vi "PicoScope6000aAdvancedTriggerPWQ.vi"(0 "handle in":i16=16384, 1 "Pulse Width Qualifier Settings":T3 {"Pulse Width Type" items=["None", "Less Than", "Greater Than", "In Range", "Out of Range"]}, 2 "Pulse Width Qualifier Trigger Properties":T1={"Channel A Trigger Properties"={"Threshold Mode"=0, "Available"=TRUE, "Direction"=2}, "Channel B Trigger Properties"={"Threshold Mode"=0, "Available"=FALSE, "Direction"=2}, "Channel C Trigger Properties"={"Threshold Mode"=0, "Available"=FALSE, "Direction"=2}, "Channel D Trigger Properties"={"Threshold Mode"=0, "Available"=FALSE, "Direction"=2}, "Channel E Trigger Properties"={"Threshold Mode"=0, "Available"=FALSE, "Direction"=2}, "Channel F Trigger Properties"={"Threshold Mode"=0, "Available"=FALSE, "Direction"=2}, "Channel G Trigger Properties"={"Threshold Mode"=0, "Available"=FALSE, "Direction"=2}, "Channel H Trigger Properties"={"Threshold Mode"=0, "Available"=FALSE, "Direction"=2}, "Port 0 Trigger Properties"={"Threshold Mode"=0, "Available"=FALSE, "Direction"=2}, "Port 1 Trigger Properties"={"Threshold Mode"=0, "Available"=FALSE, "Direction"=2}} {"Port 1 Trigger Properties"."Direction" items=["Rising"=2, "Falling"=3, "Rising Lower"=7, "Above"=0, "Below"=1, "Rising or Falling"=4, "Falling Lower"=8, "Below Lower"=6, "Above Lower"=5]; "Port 1 Trigger Properties"."Threshold Mode" items=["Level", "Window"]; "Port 0 Trigger Properties"."Direction" items=["Rising"=2, "Falling"=3, "Rising Lower"=7, "Above"=0, "Below"=1, "Rising or Falling"=4, "Falling Lower"=8, "Below Lower"=6, "Above Lower"=5]; "Port 0 Trigger Properties"."Threshold Mode" items=["Level", "Window"]; "Channel H Trigger Properties"."Direction" items=["Rising"=2, "Falling"=3, "Rising Lower"=7, "Above"=0, "Below"=1, "Rising or Falling"=4, "Falling Lower"=8, "Below Lower"=6, "Above Lower"=5]; "Channel H Trigger Properties"."Threshold Mode" items=["Level", "Window"]; "Channel G Trigger Properties"."Direction" items=["Rising"=2, "Falling"=3, "Rising Lower"=7, "Above"=0, "Below"=1, "Rising or Falling"=4, "Falling Lower"=8, "Below Lower"=6, "Above Lower"=5]; "Channel G Trigger Properties"."Threshold Mode" items=["Level", "Window"]; "Channel F Trigger Properties"."Direction" items=["Rising"=2, "Falling"=3, "Rising Lower"=7, "Above"=0, "Below"=1, "Rising or Falling"=4, "Falling Lower"=8, "Below Lower"=6, "Above Lower"=5]; "Channel F Trigger Properties"."Threshold Mode" items=["Level", "Window"]; "Channel E Trigger Properties"."Direction" items=["Rising"=2, "Falling"=3, "Rising Lower"=7, "Above"=0, "Below"=1, "Rising or Falling"=4, "Falling Lower"=8, "Below Lower"=6, "Above Lower"=5]; "Channel E Trigger Properties"."Threshold Mode" items=["Level", "Window"]; "Channel D Trigger Properties"."Direction" items=["Rising"=2, "Falling"=3, "Rising Lower"=7, "Above"=0, "Below"=1, "Rising or Falling"=4, "Falling Lower"=8, "Below Lower"=6, "Above Lower"=5]; "Channel D Trigger Properties"."Threshold Mode" items=["Level", "Window"]; "Channel C Trigger Properties"."Direction" items=["Rising"=2, "Falling"=3, "Rising Lower"=7, "Above"=0, "Below"=1, "Rising or Falling"=4, "Falling Lower"=8, "Below Lower"=6, "Above Lower"=5]; "Channel C Trigger Properties"."Threshold Mode" items=["Level", "Window"]; "Channel B Trigger Properties"."Direction" items=["Rising"=2, "Falling"=3, "Rising Lower"=7, "Above"=0, "Below"=1, "Rising or Falling"=4, "Falling Lower"=8, "Below Lower"=6, "Above Lower"=5]; "Channel B Trigger Properties"."Threshold Mode" items=["Level", "Window"]; "Channel A Trigger Properties"."Direction" items=["Rising"=2, "Falling"=3, "Rising Lower"=7, "Above"=0, "Below"=1, "Rising or Falling"=4, "Falling Lower"=8, "Below Lower"=6, "Above Lower"=5]; "Channel A Trigger Properties"."Threshold Mode" items=["Level", "Window"]}, 11 "error in":errorcluster, 13 "Pulse Width Qualifier Conditions":T2 {"Port 1" items=["Don't Care", "True", "False"]; "Channel H" items=["Don't Care", "True", "False"]; "Channel G" items=["Don't Care", "True", "False"]; "Channel F" items=["Don't Care", "True", "False"]; "Channel E" items=["Don't Care", "True", "False"]; "Aux" items=["Don't Care", "True", "False"]; "Port 0" items=["Don't Care", "True", "False"]; "Channel D" items=["Don't Care", "True", "False"]; "Channel C" items=["Don't Care", "True", "False"]; "Channel B" items=["Don't Care", "True", "False"]; "Channel A" items=["Don't Care", "True", "False"]; "Condition Logic" items=["AND", "OR", "XOR"]}) -> (4 "handle out":i16=16384, 15 "error out":errorcluster)   [LabVIEW 2010]
doc: "This sub VI is an interface for the advanced trigger features of the oscilloscope to support Pulse width qualifier (PWQ)."
uses:
  ps6000a.dll
panel:
  in  "PWQ Info Action XOR":bool=TRUE
  in  "PWQ Info Action OR":bool=TRUE
  # "For Condition Logic Suggested settings;\nFor AND, XOR logic-(parallel triggers)\nUse level-type triggers (Level or Inside/outside Window Triggers)\n\nFor OR logic- (single channel)\nUse edge types (e.g. rising, falling, entering window)"
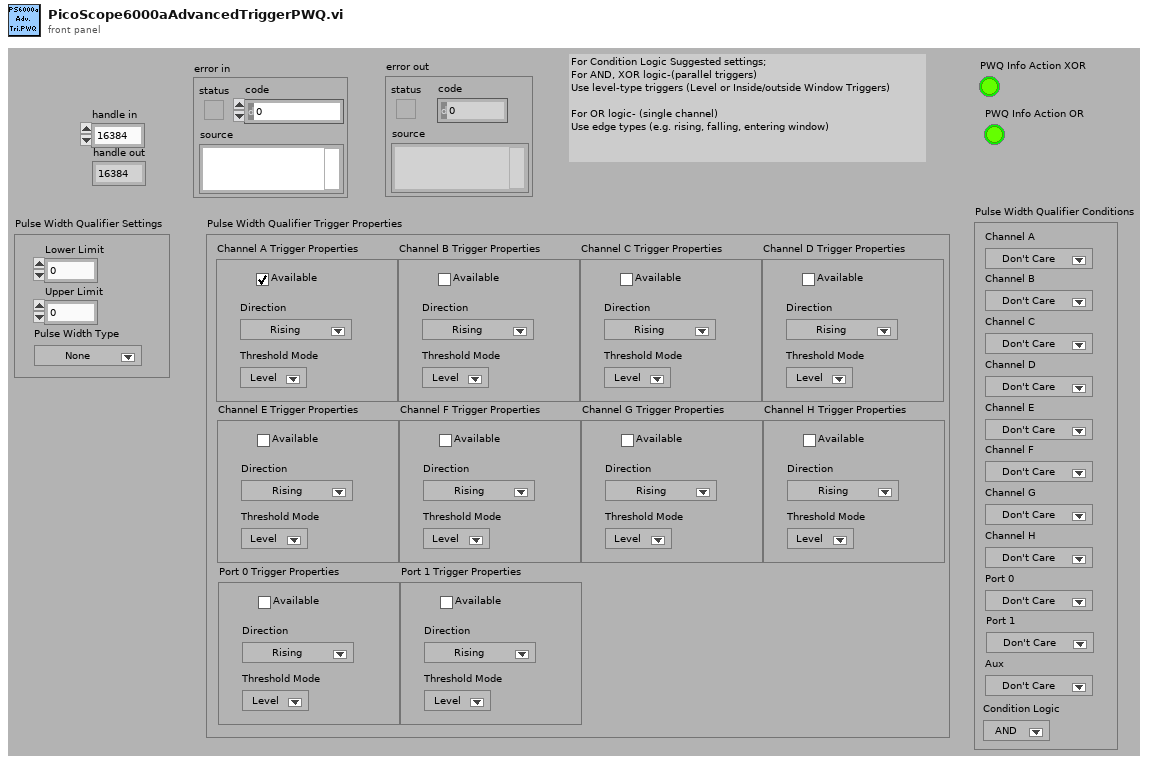
[diagram p1: front panel]
types:
  T1 = cluster{"Channel A Trigger Properties":cluster{"Threshold Mode":i32, "Available":bool, "Direction":u32}, "Channel B Trigger Properties":cluster{"Threshold Mode":i32, "Available":bool, "Direction":u32}, "Channel C Trigger Properties":cluster{"Threshold Mode":i32, "Available":bool, "Direction":u32}, "Channel D Trigger Properties":cluster{"Threshold Mode":i32, "Available":bool, "Direction":u32}, "Channel E Trigger Properties":cluster{"Threshold Mode":i32, "Available":bool, "Direction":u32}, "Channel F Trigger Properties":cluster{"Threshold Mode":i32, "Available":bool, "Direction":u32}, "Channel G Trigger Properties":cluster{"Threshold Mode":i32, "Available":bool, "Direction":u32}, "Channel H Trigger Properties":cluster{"Threshold Mode":i32, "Available":bool, "Direction":u32}, "Port 0 Trigger Properties":cluster{"Threshold Mode":i32, "Available":bool, "Direction":u32}, "Port 1 Trigger Properties":cluster{"Threshold Mode":i32, "Available":bool, "Direction":u32}}
  T2 = cluster{"Channel A":u16, "Channel B":u16, "Channel C":u16, "Channel D":u16, "Channel E":u16, "Channel F":u16, "Channel G":u16, "Channel H":u16, "Port 0":u16, "Port 1":u16, "Aux":u16, "Condition Logic":u16}
  T3 = cluster{"Lower Limit":u32, "Upper Limit":u32, "Pulse Width Type":u32}
  T4 = cluster{"status":bool, "code":u32, "source":string}
  T5 = cluster{"Threshold Mode":i32, "Available":bool, "Direction":u32}[]
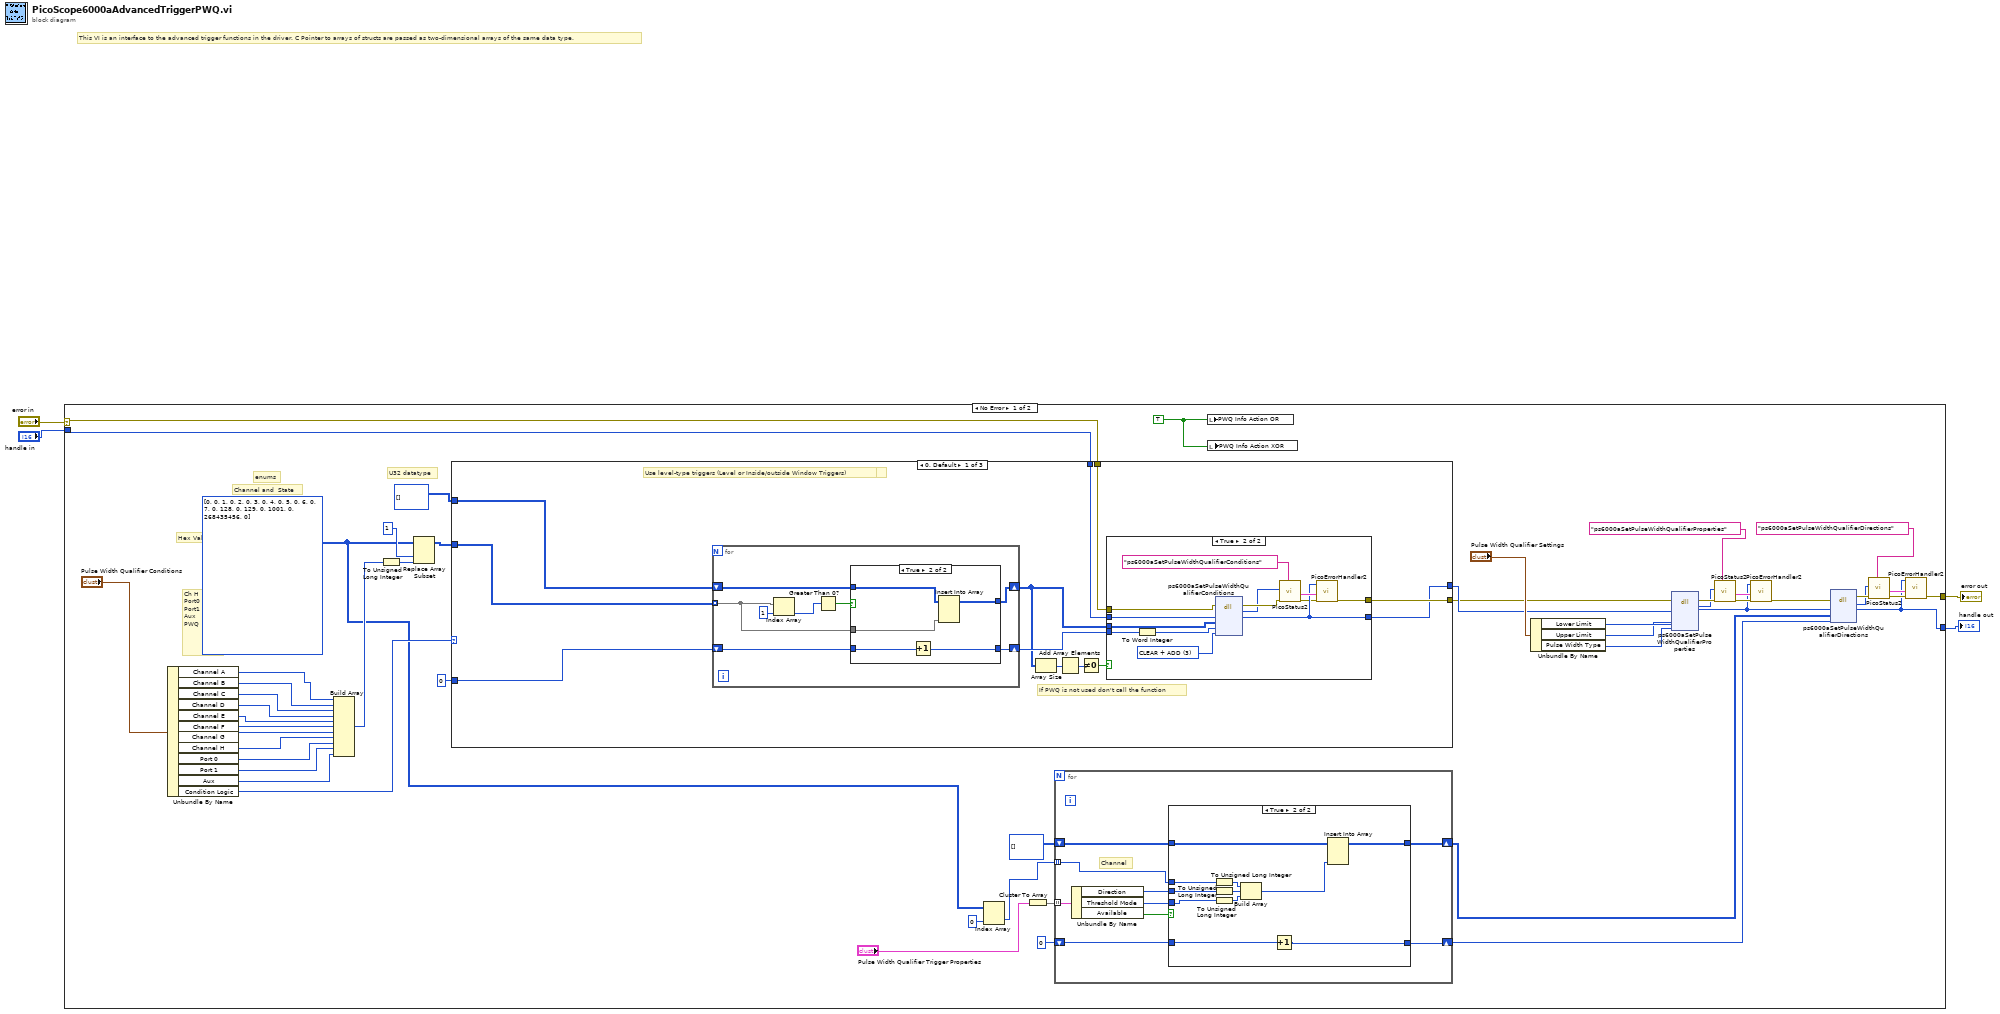
[diagram p0: block diagram]
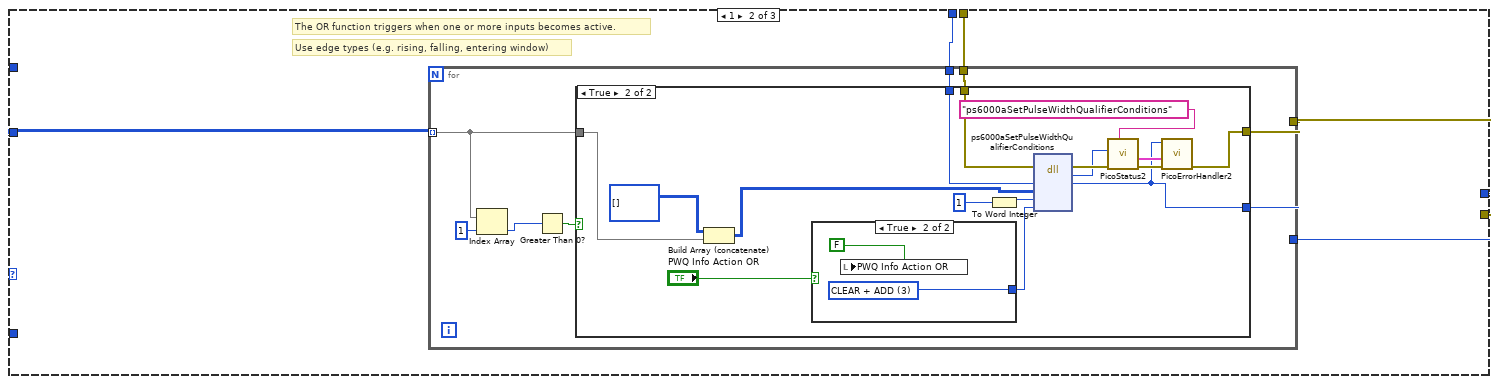
[diagram p5: hidden frame]
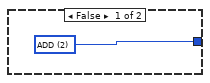
[diagram p7: hidden frame]
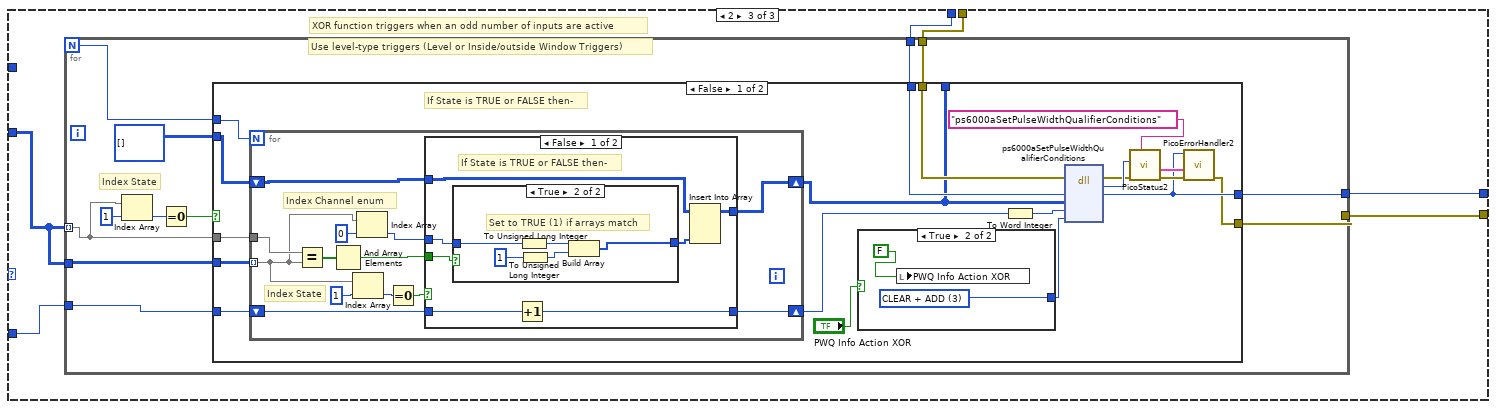
[diagram p8: hidden frame]
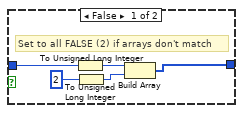
[diagram p9: hidden frame]
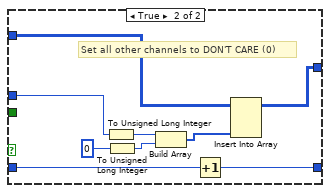
[diagram p10: hidden frame]
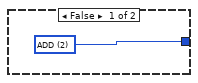
[diagram p11: hidden frame]
diagram:
  # "This VI is an interface to the advanced trigger functions in the driver. C Pointer to arrays of structs are passed as two-dimensional arrays of the same data type."
  n1 = case shown="No Error" "error in" {
    selector: "error in" -> [w20 w236]
    tunnel: "handle in" -> [w19 w237]
    tunnel: [w5 w237] -> w2
    tunnel: [w9 w236] -> w1
    frame No Error {
      w33 = TRUE ("PWQ Info Action XOR")
      w21 = u32[][] [[0, 0], [1, 0], [2, 0], [3, 0], [4, 0], [5, 0], [6, 0], [7, 0], [128, 0], [129, 0], [1001, 0], [268435456, 0]]
      # "U32 datatype"
      # "enums"
      # "Ch H\nPort0\nPort1\nAux\nPWQ"
      # "Channel and  State"
      # "Hex Values"
      n2 = Unbundle By Name("Pulse Width Qualifier Conditions") -> ("Channel A"=w43:u16, "Channel B"=w42:u16, "Channel C"=w41:u16, "Channel D"=w40:u16, "Channel E"=w39:u16, "Channel F"=w38:u16, "Channel G"=w37:u16, "Channel H"=w36:u16, "Port 0"=w35:u16, "Port 1"=w34:u16, "Aux"=w22:u16, "Condition Logic"=w23:u16)
      n3 = Build Array(w43, w42, w41, w40, w39, w38, w37, w36, w35, w34, w22) -> (w54:u16[])
      n4 = To Unsigned Long Integer(number=w54) -> (unsigned 32bit integer=w46:u32[])
      n5 = Replace Array Subset(array=w21, new element=w46, index (col)=1 ("disabled index (col)")) -> (w45:u32[][])  [unwired: 1 in]
      n6 = case shown="0, Default" w23 {
        tunnel: u32[][] [] -> [w89 _ _]
        tunnel: i16 0 -> [w88 _ w154]
        tunnel: w20 -> [w85 w124 w159]
        tunnel: w19 -> [w84 w123 w158]
        tunnel: [w83 w122 w157] -> w47
        tunnel: [w82 w121 w156] -> w48
        tunnel: w45 -> [w86 w120 w155]
        frame 0, Default {
          # "If PWQ is not used don't call the function"
          # "AND function requires both inputs to be active before it will trigger."
          # "Use level-type triggers (Level or Inside/outside Window Triggers)"
          n7 = for {
            shift-right: [w111] -> w87
            shift-left: w88 -> [w110]
            shift-right: [w109] -> w81
            shift-left: w89 -> [w112]
            tunnel: w86 -> [w107] mode=indexing
            n8 = Index Array(array=w107, index=1) -> (element=w106:u32)
            n9 = Greater Than 0?(x=w106) -> (x > 0?=w108:bool)
            n10 = case shown="True" w108 {
              tunnel: w112 -> [w114 w119]
              tunnel: [w114 w118] -> w109
              tunnel: [w113 w117] -> w111
              tunnel: w110 -> [w113 w116]
              tunnel: w107 -> [_ w115]
              frame False {
              }
              frame True {
                n11 = Increment(x=w116) -> (x+1=w117:i16)
                n12 = Insert Into Array(array=w119, new element=w115) -> (w118:u32[][])  [unwired: 2 in]
              }
            }
          }
          n13 = Array Size(array=w81) -> (size(s)=w79:i32[])
          n14 = Add Array Elements(numeric array=w79) -> (sum=w80:i32)
          n15 = Not Equal To 0?(x=w80) -> (x != 0?=w78:bool)
          n16 = case shown="True" w78 {
            tunnel: w87 -> [_ w104]
            tunnel: w85 -> [w91 w103]
            tunnel: w84 -> [w90 w102]
            tunnel: w81 -> [_ w99]
            tunnel: [w91 w96] -> w83
            tunnel: [w90 w93] -> w82
            frame False {
            }
            frame True {
              w101 = u32 3 items=["CLEAR + ADD"=3, "CLEAR"=1, "ADD"=2] ("Condition Action")
              n17 = To Word Integer(number=w104) -> (16bit integer=w100:i16)
              n18 = dll-call lib="ps6000a.dll" fn="ps6000aSetPulseWidthQualifierConditions" ("ps3000.dll:_ps3000_open_unit@0")(error in=w103, "handle"=w102, "conditions"=w99, "nConditions"=w100, "action"=w101) -> (error out=w97:errorcluster, "PICO_STATUS"=w95:u32, "handle"=w93:i16)  [unwired: 5 in, 1 out]
              n19 = call "PicoStatus2.vi"("PICO source"="ps6000aSetPulseWidthQualifierConditions" ("source"), "Error in"=w97, "PICO STATUS"=w95) -> ("error out"=w92:errorcluster, "PICO_STATUS out"=w98:T4)  [unwired: 5 in]
              n20 = call "PicoErrorHandler2.vi"("error in (no error)"=w92, "PICO_STATUS in"=w98, "handle In"=w93) -> ("error out"=w96:errorcluster)  [unwired: 8 in]
            }
          }
        }
        frame 1 {
          # "Use edge types (e.g. rising, falling, entering window)"
          # "The OR function triggers when one or more inputs becomes active."
          n21 = for {
            tunnel: w124 -> [w132]
            tunnel: w123 -> [w131]
            tunnel: [w130] -> w122
            tunnel: [w129] -> w121
            tunnel: w120 -> [w127] mode=indexing
            n22 = Index Array(array=w127, index=1) -> (element=w126:u32)
            n23 = Greater Than 0?(x=w126) -> (x > 0?=w125:bool)
            n24 = case shown="True" w125 {
              tunnel: w132 -> [w133 w149]
              tunnel: w131 -> [w134 w148]
              tunnel: [w133 w138] -> w130
              tunnel: [w134 w135] -> w129
              tunnel: w127 -> [_ w142]
              frame False {
              }
              frame True {
                n25 = Build Array (concatenate)(u32[][] [], w142) -> (w144:u32[][])
                n26 = case shown="True" "PWQ Info Action OR" {
                  tunnel: [w151 w153] -> w147
                  frame False {
                    w151 = u32 2 items=["CLEAR"=1, "ADD"=2, "CLEAR + ADD"=3] ("Condition Action")
                  }
                  frame True {
                    w153 = u32 3 items=["CLEAR"=1, "ADD"=2, "CLEAR + ADD"=3] ("Condition Action")
                    n27 = local write "PWQ Info Action OR"(FALSE ("Boolean")) -> ()
                  }
                }
                n28 = To Word Integer(number=i16 1) -> (16bit integer=w150:i16)
                n29 = dll-call lib="ps6000a.dll" fn="ps6000aSetPulseWidthQualifierConditions" ("ps3000.dll:_ps3000_open_unit@0")(error in=w149, "handle"=w148, "conditions"=w144, "nConditions"=w150, "action"=w147) -> (error out=w139:errorcluster, "PICO_STATUS"=w136:u32, "handle"=w135:i16)  [unwired: 5 in, 1 out]
                n30 = call "PicoStatus2.vi"("PICO source"="ps6000aSetPulseWidthQualifierConditions" ("source"), "Error in"=w139, "PICO STATUS"=w136) -> ("error out"=w140:errorcluster, "PICO_STATUS out"=w141:T4)  [unwired: 5 in]
                n31 = call "PicoErrorHandler2.vi"("error in (no error)"=w140, "PICO_STATUS in"=w141, "handle In"=w135) -> ("error out"=w138:errorcluster)  [unwired: 8 in]
              }
            }
          }
        }
        frame 2 {
          # "Use level-type triggers (Level or Inside/outside Window Triggers)"
          # "XOR function triggers when an odd number of inputs are active"
          n32 = for {
            N -> [w167]
            tunnel: w159 -> [w171]
            tunnel: w158 -> [w170]
            tunnel: [w169] -> w157
            tunnel: [w168] -> w156
            tunnel: w155 -> [w161] mode=indexing
            tunnel: w155 -> [w164]
            tunnel: w154 -> [w165]
            # "Index State"
            n33 = Index Array(array=w161, index=1) -> (element=w162:u32)
            n34 = Equal To 0?(x=w162) -> (x = 0?=w160:bool)
            n35 = case shown="False" w160 {
              tunnel: w171 -> [w190 w233]
              tunnel: w170 -> [w189 w234]
              tunnel: [w175 w233] -> w169
              tunnel: [w176 w234] -> w168
              tunnel: [w187 w235] -> _
              tunnel: w167 -> [w186 _]
              tunnel: u32[][] [] -> [w185 w235]
              tunnel: w165 -> [w184 _]
              tunnel: w164 -> [w183 _]
              tunnel: w161 -> [w182 _]
              frame False {
                # "If State is TRUE or FALSE then-"
                n36 = for {
                  N: w186 -> [_]
                  shift-right: [w202] -> w188
                  shift-left: w184 -> [w203]
                  shift-right: [w191] -> w187
                  shift-left: w185 -> [w192]
                  tunnel: w182 -> [w199]
                  tunnel: w183 -> [w195] mode=indexing
                  # "Index State"
                  # "Index Channel enum"
                  n37 = Equal?(x=w199, y=w195) -> (x = y?=w193:bool[])
                  n38 = And Array Elements(Boolean array=w193) -> (logical AND=w198:bool)
                  n39 = Index Array(array=w195, index=1) -> (element=w196:u32)
                  n40 = Index Array(array=w195, index=0) -> (element=w200:u32)
                  n41 = Equal To 0?(x=w196) -> (x = 0?=w194:bool)
                  n42 = case shown="False" w194 {
                    tunnel: w203 -> [w210 w221]
                    tunnel: [w209 w222] -> w202
                    tunnel: w200 -> [w208 w225]
                    tunnel: w198 -> [w207 _]
                    tunnel: w192 -> [w206 w224]
                    tunnel: [w204 w223] -> w191
                    frame False {
                      # "If State is TRUE or FALSE then-"
                      n43 = case shown="True" w207 {
                        tunnel: [w215 w220] -> w205
                        tunnel: w208 -> [w214 w219]
                        frame False {
                          # "Set to all FALSE (2) if arrays don't match"
                          n44 = To Unsigned Long Integer(number=w214) -> (unsigned 32bit integer=w212:u32)
                          n45 = To Unsigned Long Integer(number=u32 2) -> (unsigned 32bit integer=w213:u32)
                          n46 = Build Array(w212, w213) -> (w215:u32[])
                        }
                        frame True {
                          # "Set to TRUE (1) if arrays match"
                          n47 = To Unsigned Long Integer(number=w219) -> (unsigned 32bit integer=w217:u32)
                          n48 = To Unsigned Long Integer(number=u32 1) -> (unsigned 32bit integer=w218:u32)
                          n49 = Build Array(w217, w218) -> (w220:u32[])
                        }
                      }
                      n50 = Increment(x=w210) -> (x+1=w209:i16)
                      n51 = Insert Into Array(array=w206, new element=w205) -> (w204:u32[][])  [unwired: 2 in]
                    }
                    frame True {
                      # "Set all other channels to DON'T CARE (0)"
                      n52 = To Unsigned Long Integer(number=w225) -> (unsigned 32bit integer=w227:u32)
                      n53 = To Unsigned Long Integer(number=u32 0) -> (unsigned 32bit integer=w228:u32)
                      n54 = Build Array(w227, w228) -> (w229:u32[])
                      n55 = Increment(x=w221) -> (x+1=w222:i16)
                      n56 = Insert Into Array(array=w224, new element=w229) -> (w223:u32[][])  [unwired: 2 in]
                    }
                  }
                }
                n57 = case shown="True" "PWQ Info Action XOR" {
                  tunnel: [w230 w232] -> w179
                  frame False {
                    w230 = u32 2 items=["CLEAR + ADD"=3, "CLEAR"=1, "ADD"=2] ("Condition Action")
                  }
                  frame True {
                    w232 = u32 3 items=["CLEAR + ADD"=3, "CLEAR"=1, "ADD"=2] ("Condition Action")
                    n58 = local write "PWQ Info Action XOR"(FALSE ("Boolean")) -> ()
                  }
                }
                n59 = To Word Integer(number=w188) -> (16bit integer=w181:i16)
                n60 = dll-call lib="ps6000a.dll" fn="ps6000aSetPulseWidthQualifierConditions" ("ps3000.dll:_ps3000_open_unit@0")(error in=w190, "handle"=w189, "conditions"=w187, "nConditions"=w181, "action"=w179) -> (error out=w172:errorcluster, "PICO_STATUS"=w173:u32, "handle"=w176:i16)  [unwired: 5 in, 1 out]
                n61 = call "PicoStatus2.vi"("PICO source"="ps6000aSetPulseWidthQualifierConditions" ("source"), "Error in"=w172, "PICO STATUS"=w173) -> ("error out"=w177:errorcluster, "PICO_STATUS out"=w178:T4)  [unwired: 5 in]
                n62 = call "PicoErrorHandler2.vi"("error in (no error)"=w177, "PICO_STATUS in"=w178, "handle In"=w176) -> ("error out"=w175:errorcluster)  [unwired: 8 in]
              }
              frame True {
              }
            }
          }
        }
      }
      n63 = Index Array(array=w21, index (col)=0 ("disabled index (col)")) -> (element=w24:u32[])  [unwired: 1 in]
      n64 = Cluster To Array(cluster="Pulse Width Qualifier Trigger Properties") -> (array=w30:T5)
      n65 = for {
        tunnel: w30 -> [w64] mode=indexing
        shift-right: [w59] -> w28
        shift-left: u32[][] [] -> [w60]
        shift-right: [w57] -> w26
        shift-left: i16 0 ("nDirections") -> [w58]
        tunnel: w24 -> [w56] mode=indexing
        # "Channel"
        n66 = Unbundle By Name(w64) -> ("Direction"=w62:u32, "Threshold Mode"=w61:i32, "Available"=w63:bool)
        n67 = case shown="True" w63 {
          tunnel: w56 -> [_ w73]
          tunnel: w62 -> [_ w72]
          tunnel: w61 -> [_ w71]
          tunnel: w60 -> [w66 w70]
          tunnel: [w66 w69] -> w59
          tunnel: [w65 w68] -> w57
          tunnel: w58 -> [w65 w67]
          frame False {
          }
          frame True {
            n68 = To Unsigned Long Integer(number=w73) -> (unsigned 32bit integer=w75:u32)
            n69 = To Unsigned Long Integer(number=w72) -> (unsigned 32bit integer=w76:u32)
            n70 = To Unsigned Long Integer(number=w71) -> (unsigned 32bit integer=w74:u32)
            n71 = Build Array(w75, w76, w74) -> (w77:u32[])
            n72 = Increment(x=w67) -> (x+1=w68:i16)
            n73 = Insert Into Array(array=w70, new element=w77) -> (w69:u32[][])  [unwired: 2 in]
          }
        }
      }
      n74 = local write "PWQ Info Action OR"(w33) -> ()
      n75 = local write "PWQ Info Action XOR"(w33) -> ()
      n76 = Unbundle By Name("Pulse Width Qualifier Settings") -> ("Lower Limit"=w53:u32, "Upper Limit"=w52:u32, "Pulse Width Type"=w51:u32)
      n77 = dll-call lib="ps6000a.dll" fn="ps6000aSetPulseWidthQualifierProperties" ("ps3000.dll:_ps3000_open_unit@0")(error in=w47, "handle"=w48, "lower"=w53, "upper"=w52, "type"=w51) -> (error out=w14:errorcluster, "PICO_STATUS"=w12:u32, "handle"=w11:i16)  [unwired: 5 in, 1 out]
      n78 = call "PicoStatus2.vi"("PICO source"="ps6000aSetPulseWidthQualifierProperties" ("source"), "Error in"=w14, "PICO STATUS"=w12) -> ("error out"=w17:errorcluster, "PICO_STATUS out"=w18:T4)  [unwired: 5 in]
      n79 = call "PicoErrorHandler2.vi"("error in (no error)"=w17, "PICO_STATUS in"=w18, "handle In"=w11) -> ("error out"=w10:errorcluster)  [unwired: 8 in]
      n80 = dll-call lib="ps6000a.dll" fn="ps6000aSetPulseWidthQualifierDirections" ("ps3000.dll:_ps3000_open_unit@0")(error in=w10, "handle"=w11, "directions"=w28, "nDirections"=w26) -> (error out=w8:errorcluster, "PICO_STATUS"=w6:u32, "handle"=w5:i16)  [unwired: 4 in, 1 out]
      n81 = call "PicoStatus2.vi"("PICO source"="ps6000aSetPulseWidthQualifierDirections" ("source"), "Error in"=w8, "PICO STATUS"=w6) -> ("error out"=w15:errorcluster, "PICO_STATUS out"=w16:T4)  [unwired: 5 in]
      n82 = call "PicoErrorHandler2.vi"("error in (no error)"=w15, "PICO_STATUS in"=w16, "handle In"=w5) -> ("error out"=w9:errorcluster)  [unwired: 8 in]
    }
    frame Error {
    }
  }
  "handle out" <- w2
  "error out" <- w1
